vi "Import Parameters Configuration to New AIM ARINC 429 Custom Device.vi"(7 "Base System Definition File":path=path "Support/Base.nivssdf", 9 "Parameters Configuration File":path=path "Support/Parameters in Scheduled and Dynamic Labels.xml", 11 "Output System Definition File":path=path "Support/Imported AIM ARINC 429.nivssdf") -> (3 "AIM ARINC 429 System Definition":path)   [LabVIEW 2020]
doc: "Overview: Demonstrates using the Ballard ARINC 429 scripting API to configure the custom device by importing a parameters configuration file. \n\nInstructions:\n1. Specify the Parameters Configuration File. This parameters configuration file must be consistent with the schema published on the GitHub repo (https://github.com/ni/niveristand-ballard-arinc429-custom-device/blob/main/Docs/Parameters%20XML%20File/ARINC429_Parameters_XML_Schema.xsd). For successful deployment, the parameters configuration file must also be consistent with the hardware configuration file.\n2. Specify the Hardware Configuration File. The hardware configuration file must be consistent with the schema installed by the Ballard hardware driver at C:\\Program Files (x86)\\Astronics Ballard Technology LabVIEW Driver\\Help\\index.html.\n3. (VeriStand) Optionally, you may open the Ballard ARINC 429 System Definition in VeriStand, configure the PXI Linux RT Target, and deploy the scripted system definition to perform avionics bus communications with Ballard ARINC 429 hardware."
uses:
  <vilib>/addons/VeriStand Custom Device Scripting APIs/AIM ARINC 429/Shared/Device Parameters.ctl
  NationalInstruments.VeriStand.SystemDefinitionAPI
  AIM ARINC 429 Scripting Examples.lvlib
  <vilib>/addons/VeriStand Custom Device Scripting APIs/AIM ARINC 429/Scripting/AIM/AIM ARINC 429 Scripting.lvlib
panel:
  # "Overview: Demonstrates using the AIM ARINC 429 scripting API to configure the custom device by importing a parameters configuration file. \n\nInstructions:\n1. Specify the Parameters Configuration File. This parameters configuration file must be consistent with the schema published on the GitHub repo (https://github.com/ni/niveristand-aim-arinc429-custom-device/blob/main/Docs/Parameters%20XML%20File/ARINC429_Parameters_XML_Schema.xsd).\n3. (VeriStand) Optionally, you may open the AIM ARINC 429 System Definition in VeriStand, configure the PXI Linux RT Target, and deploy the scripted system definition to perform avionics bus communications with AIM ARINC 429 hardware."
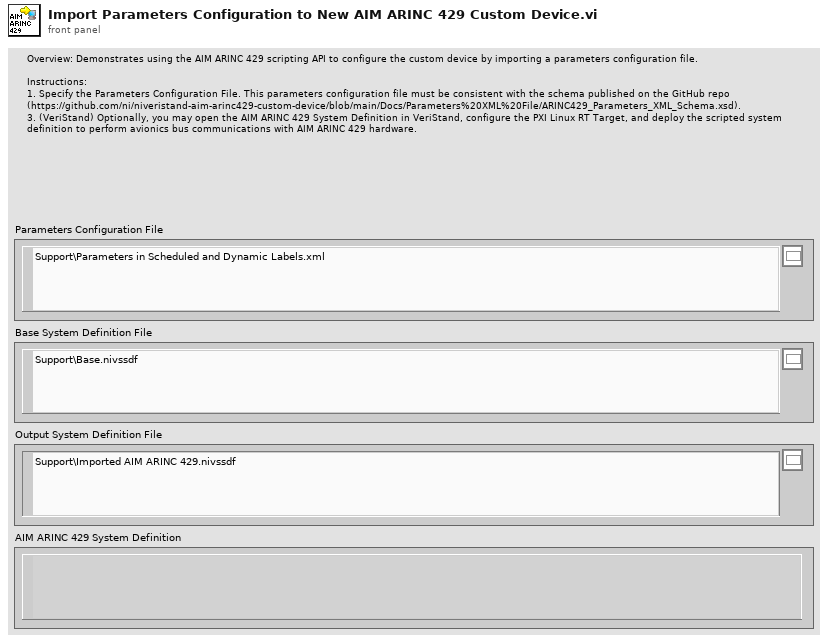
[diagram p1: front panel]
types:
  T1 = typedef "Device Parameters.ctl" = cluster{"pxi slot":u8}
  T2 = typedef "Custom Device API.lvlib/Custom Device Item Ref.ctl" = u64
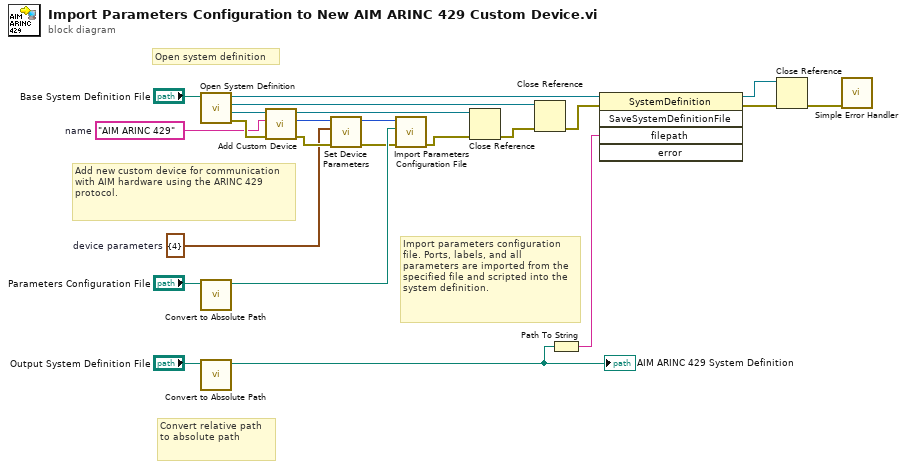
[diagram p0: block diagram]
diagram:
  w1 = T1 {"pxi slot"=4}  # device parameters
  w11 = "AIM ARINC 429"  # name
  # "Import parameters configuration file. Ports, labels, and all parameters are imported from the specified file and scripted into the system definition."
  # "Add new custom device for communication with AIM hardware using the ARINC 429 protocol."
  # "Convert relative path to absolute path"
  # "Open system definition"
  # "8."
  n1 = call "Open System Definition.vi"("system definition file"="Base System Definition File") -> ("error out"=w12:errorcluster, "target"=w13:refnum<k24>, "root"=w15:refnum<k24>, "system definition"=w16:refnum<k24>)  [unwired: 7 in]
  n2 = call "Convert to Absolute Path.vi"("system definition file"="Parameters Configuration File") -> ("absolute path"=w9:path)  [unwired: 10 in]
  n3 = call "Convert to Absolute Path.vi"("system definition file"="Output System Definition File") -> ("absolute path"=w6:path)  [unwired: 10 in]
  "AIM ARINC 429 System Definition" <- w6
  n4 = call <vilib>:"Add Custom Device.vi"("error in"=w12, "name"=w11, "target"=w13) -> ("error out"=w3:errorcluster, "AIM ARINC 429 custom device"=w5:T2, "target out"=w7:refnum<k24>)  [unwired: 6 in]
  n5 = call <vilib>:"Set Device Parameters.vi"("error in"=w3, "device parameters"=w1, "custom device"=w5) -> ("error out"=w2:errorcluster, "custom device ref out"=w4:T2)  [unwired: 7 in]
  n6 = call <vilib>:"Import Parameters Configuration File.vi"("error in"=w2, "parameters configuration file path"=w9, "custom device ref"=w4) -> ("error out"=w8:errorcluster)  [unwired: 7 in, 1 out]
  n7 = Close Reference(reference=w7, error in (no error)=w8) -> (error out=w14:errorcluster)
  n8 = Close Reference(reference=w15, error in (no error)=w14) -> (error out=w19:errorcluster)
  n9 = Path To String(path=w6) -> (string=w22:string)
  n10 = invoke class="SystemDefinition" method="SaveSystemDefinitionFile"(reference=w16, error in=w19, "filepath"=w22) -> (reference out=w20:refnum<k24>, error out=w21:errorcluster)  [unwired: 2 in, 3 out]
  n11 = Close Reference(reference=w20, error in (no error)=w21) -> (error out=w18:errorcluster)
  n12 = call <vilib>:"Simple Error Handler.vi"("error in (no error)"=w18) -> ()  [unwired: 1 in, 8 out]
